vi "Merge Error Wire.vi"(1 "Local Context (None)":string, 2 "error in (no error)":errorcluster, 3 "Call Chain (F)":bool, 5 "MultiErrors in":refnum<class "MultiErrors.lvclass">) -> (6 "MultiErrors out":refnum<class "MultiErrors.lvclass">)   [LabVIEW 2020, in "VolatusErrorUtilities.lvlib" / "MultiErrors.lvclass"]
uses:
  MultiErrors.lvclass
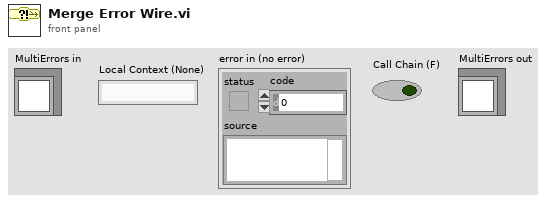
[diagram p1: front panel]
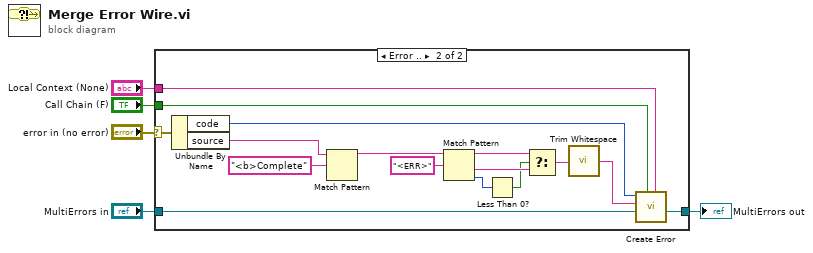
[diagram p0: block diagram]
diagram:
  n1 = case shown="Error .." "error in (no error)" {
    selector: "error in (no error)" -> [_ w21]
    tunnel: "MultiErrors in" -> [w6 w19]
    tunnel: "Call Chain (F)" -> [_ w22]
    tunnel: [w6 w7] -> w2
    tunnel: "Local Context (None)" -> [_ w8]
    frame No Error {
    }
    frame Error {
      n2 = Unbundle By Name(w21) -> ("code"=w20:i32, "source"=w18:string)
      n3 = Match Pattern(string=w18, regular expression="<b>Complete") -> (before substring=w15:string)  [unwired: 1 in, 3 out]
      n4 = Match Pattern(string=w15, regular expression="<ERR>") -> (before substring=w12:string, after substring=w11:string, offset past match=w13:i32)  [unwired: 1 in, 1 out]
      n5 = Less Than 0?(x=w13) -> (x < 0?=w10:bool)
      n6 = Select(t=w12, s=w10, f=w11) -> (s? t:f=w9:string)
      n7 = call <vilib>:"Trim Whitespace.vi"("string"=w9) -> ("trimmed string"=w16:string)  [unwired: 1 in]
      n8 = call "Create Error.vi"("Local Context (None)"=w8, "Call Chain (F)"=w22, "MultiErrors in"=w19, "Message"=w16, "Code"=w20) -> ("MultiErrors out"=w7:refnum<class "MultiErrors.lvclass">)  [unwired: 6 in]
    }
  }
  "MultiErrors out" <- w2
